vi "Set Cluster variables(SubVI).vi"(10 "In new":dbl, 11 "In original":dbl) -> (3 "Out":dbl)   [LabVIEW 2014]
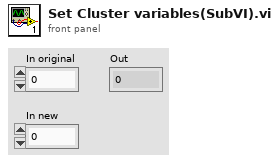
[diagram p1: front panel]
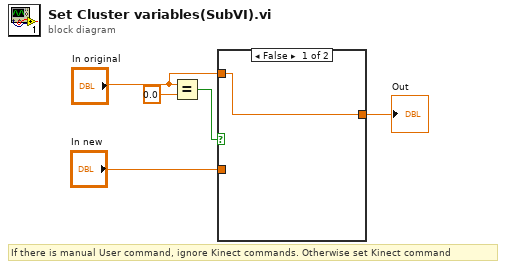
[diagram p0: block diagram]
diagram:
  # "If there is manual User command, ignore Kinect commands. Otherwise set Kinect command"
  n1 = Equal?(x="In original", y=0.0) -> (x = y?=w2:bool)
  n2 = case shown="False" w2 {
    tunnel: "In new" -> [_ w7]
    tunnel: "In original" -> [w6 _]
    tunnel: [w6 w7] -> w5
    frame False {
    }
    frame True {
    }
  }
  "Out" <- w5
